vi "Generate Trace for New Network Endpoint Client.vi"(8 "Device IPs":string[](array[string]), 9 "Port":string, 10 "IP or Stream Name":string) -> ()   [LabVIEW 2020]
doc: "Generates a DETT User Generated Trace for a network endpoint being newly launched."
uses:
  <resource>/AFDebug/AF Debug.lvlib
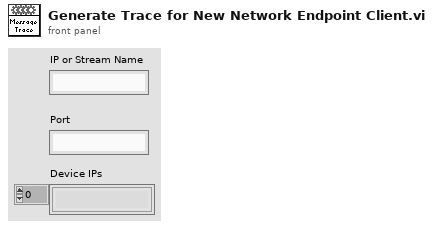
[diagram p1: front panel]
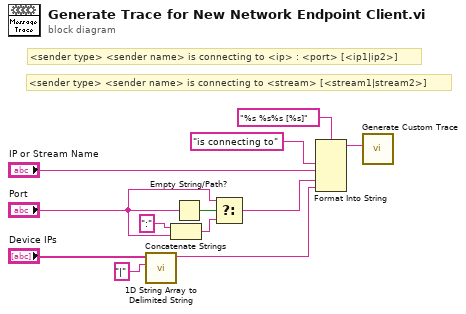
[diagram p0: block diagram]
diagram:
  # "<sender type> <sender name> is connecting to <ip> : <port> [<ip1|ip2>]"
  # "<sender type> <sender name> is connecting to <stream> [<stream1|stream2>]"
  n1 = call-poly <vilib>:"1D String Array to Delimited String.vi"("delimiter"="|", "string array"="Device IPs") -> ("delimited string"=w2:string)  [unwired: 9 in]
  n2 = Concatenate Strings(":" ("string"), "Port") -> (w7:string)
  n3 = Empty String/Path?(string/path="Port") -> (empty?=w8:bool)
  n4 = Select(t="Port", s=w8, f=w7) -> (s? t:f=w6:string)
  n5 = Format Into String(format string="%s %s%s [%s]", "is connecting to" ("input 3"), "IP or Stream Name", w6, w2) -> (resulting string=w10:string)  [unwired: 2 in, 1 out]
  n6 = call <resource>:"Generate Custom Trace.vi"("Custom Action"=w10) -> ()  [unwired: 11 in]
